vi "Get Custom Device Ref.vi"(8 "error in":errorcluster, 9 "Custom Device GUID_Disabled":string, 10 "Custom Device GUID":string, 11 "Section Ptr":T1 format="%.0x") -> (0 "error out":errorcluster, 2 "Custom Device Ref":T1 format="%.0x", 3 "Section Ref out":T1 format="%.0x")   [LabVIEW 2025, in "Protection and Counter Addon System Explorer.lvlib"]
uses:
  Protection and Counter Addon System Explorer.lvlib
  <vilib>/NI VeriStand/Custom Device API/Custom Device Item Ref.ctl
  <vilib>/NI VeriStand/Custom Device Tools/Custom Device Utility Library/Search Direction.ctl
  <vilib>/NI VeriStand/Custom Device Tools/Custom Device Utility Library/NI VeriStand - Search for Item by GUID.vi
  <vilib>/NI VeriStand/Custom Device Tools/Custom Device Utility Library/Custom Device Utility Library.lvlib
  <vilib>/NI VeriStand/Custom Device API/Custom Device API.lvlib
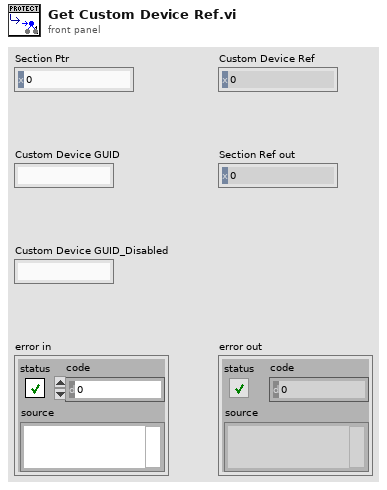
[diagram p1: front panel]
types:
  T1 = typedef "Custom Device API.lvlib/Custom Device Item Ref.ctl" = u64
  T2 = typedef "Custom Device Utility Library.lvlib/Search Direction.ctl" = enum16{"Down", "Up"}
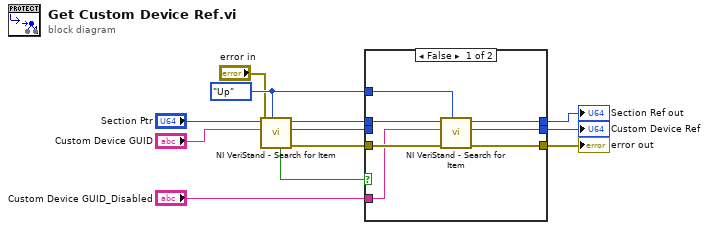
[diagram p0: block diagram]
diagram:
  w2 = Search_Direction."Up" ("Direction (Down)")
  n1 = call-poly <vilib>:"NI VeriStand - Search for Item.vi"("Direction (Down)"=w2, "error in"="error in", "Item GUID"="Custom Device GUID", "Section Ref in"="Section Ptr") -> ("error out"=w3:errorcluster, "Item Ref"=w10:T1, "Section Ref out"=w4:T1, "Found"=w7:bool)  [unwired: 4 in]
  n2 = case shown="False" w7 {
    tunnel: w2 -> [w19 _]
    tunnel: w3 -> [w18 w22]
    tunnel: w4 -> [w17 w21]
    tunnel: [w16 w21] -> w6
    tunnel: "Custom Device GUID_Disabled" -> [w15 _]
    tunnel: [w14 w20] -> w11
    tunnel: [w13 w22] -> w12
    tunnel: w10 -> [_ w20]
    frame False {
      n3 = call-poly <vilib>:"NI VeriStand - Search for Item.vi"("Direction (Down)"=w19, "error in"=w18, "Item GUID"=w15, "Section Ref in"=w17) -> ("error out"=w13:errorcluster, "Item Ref"=w14:T1, "Section Ref out"=w16:T1)  [unwired: 4 in, 1 out]
    }
    frame True {
    }
  }
  "error out" <- w12
  "Custom Device Ref" <- w11
  "Section Ref out" <- w6
